vi "LCD_I2C_Ex.vi"() -> ()   [LabVIEW 2026]
panel:
  in  "Fila":u8
  in  "Columna":u8
  in  "String":string
  in  "Direccion":u8 format="%x"
  out "respuesta":string
  in  "VISA resource name":refnum<visa-resource-name>
  in  "Stop Button":bool
  out "error out":errorcluster
  # "Ejemplo: LCD I2C"
  # "Descripción: Escribe en una pantalla LCD I2C de 16x2"
  # "Configuracion"
  # "Indicadores"
  # "Control"
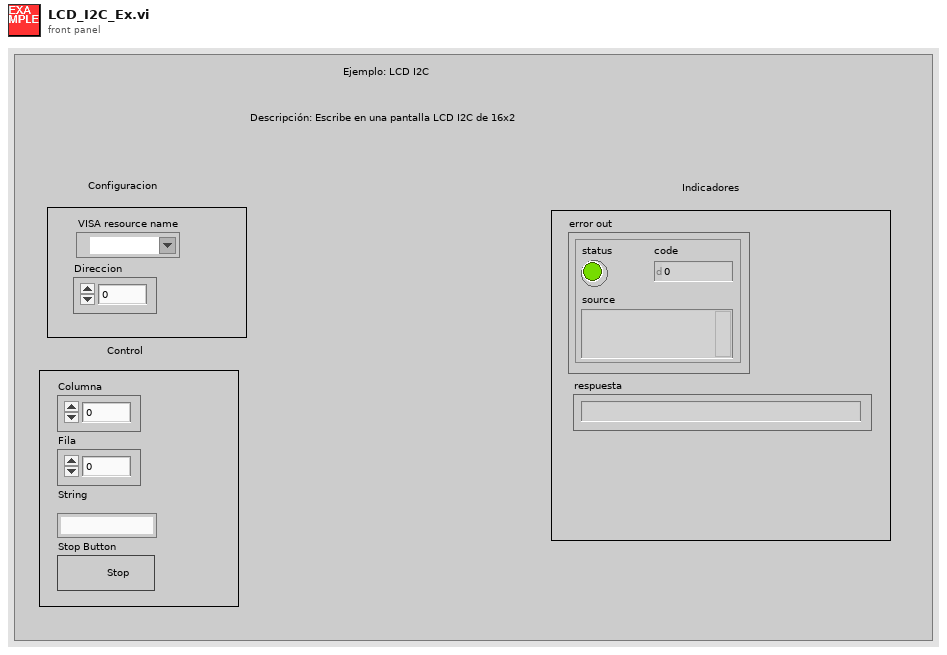
[diagram p1: front panel]
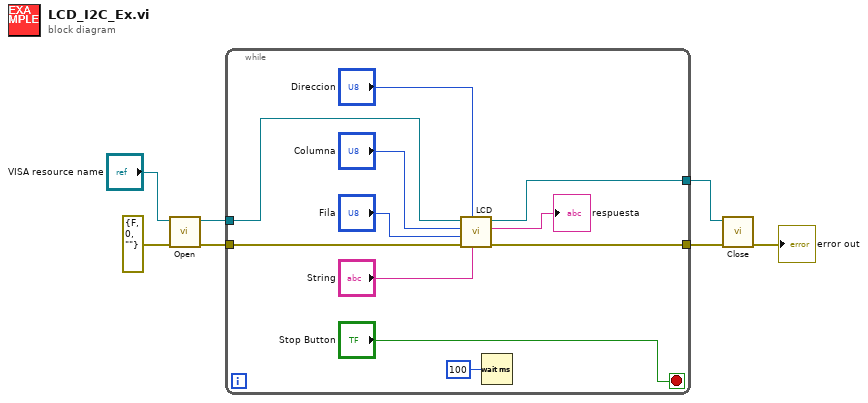
[diagram p0: block diagram]
diagram:
  n1 = call "Open.vi"("error in (no error)"=errorcluster {"status"=FALSE, "code"=0, "source"=""}, "VISA resource name"="VISA resource name") -> ("error out"=w7:errorcluster, "VISA resource name out"=w6:refnum<visa-resource-name>)  [unwired: 8 in]
  n2 = while {
    tunnel: w6 -> [w16]
    tunnel: w7 -> [w15]
    tunnel: [w14] -> w2
    tunnel: [w13] -> w1
    stop <- "Stop Button" stop-if-true
    n3 = call "LCD.vi"("String"="String", "Direccion"="Direccion", "error in (no error)"=w15, "Fila"="Fila", "Columna"="Columna", "VISA resource name"=w16) -> ("error out"=w14:errorcluster, "respuesta"=→"respuesta":string, "VISA resource name out"=w13:refnum<visa-resource-name>)  [unwired: 3 in]
    n4 = Wait (ms)(milliseconds to wait=u32 100) -> ()  [unwired: 1 out]
  }
  n5 = call "Close.vi"("error in (no error)"=w2, "VISA resource name"=w1) -> ("error out"=→"error out":errorcluster)  [unwired: 9 in]
